vi "Initialize.vi"(8 "error in":errorcluster, 9 "Python Module":path, 10 "Output Folder":path, 11 "G-CLI Runner in":refnum<class "Runner.lvclass">) -> (0 "error out":errorcluster, 3 "G-CLI Runner out":refnum<class "Runner.lvclass">)   [LabVIEW 2026, in "Runner.lvlib" / "Runner.lvclass"]
doc: "Initialize runner."
uses:
  Runner.lvclass
  Runner.lvclass/Runner.ctl
  Interfaces/ILogger/ILogger Messages/Log Msg/Log Msg.lvclass/Log Msg.ctl
  <vilib>/ActorFramework/Message Enqueuer/Message Enqueuer.lvclass/Message Enqueuer.ctl
  <vilib>/ActorFramework/Message Enqueuer/Enqueue.vi
  Interfaces/ILogger/ILogger Messages/Log Msg/Log Msg.lvclass
  <vilib>/ActorFramework/Message Priority Queue/Priority Enqueue.vi
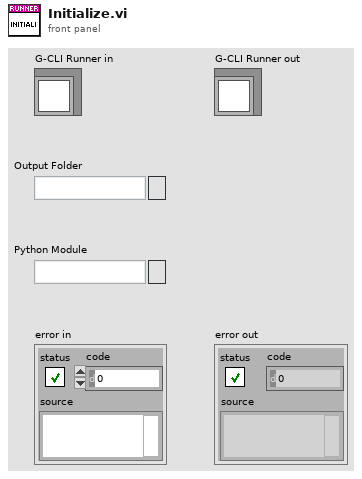
[diagram p1: front panel]
types:
  T1 = typedef "Paths And Strings--cluster.ctl" = cluster{"Project File":path, "Project Folder":path, "Module Name":string}
  T2 = typedef "Log Entry--cluster.ctl" = cluster{"Time":timestamp, "Message":string}
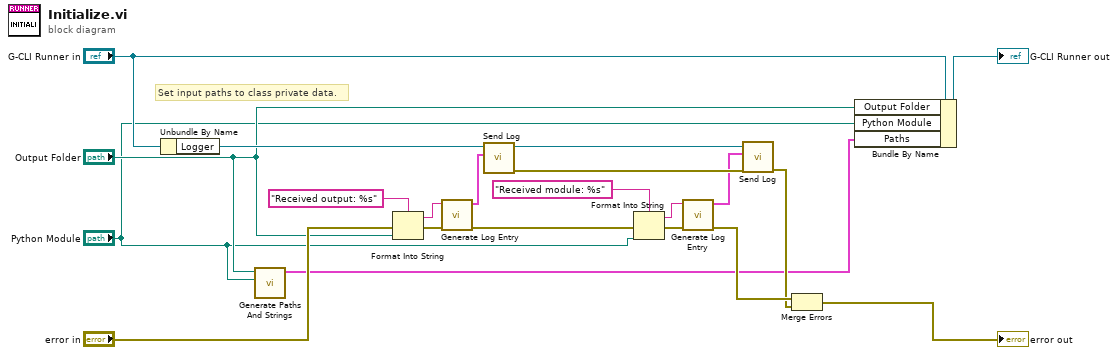
[diagram p0: block diagram]
diagram:
  # "Set input paths to class private data."
  n1 = Unbundle By Name("G-CLI Runner in") -> ("Logger"=w11:refnum<class "Message Enqueuer.lvclass">)
  n2 = call "Generate Paths And Strings.vi"("Python Module"="Python Module", "Output Folder"="Output Folder") -> ("Paths"=w1:T1)  [unwired: 9 in]
  n3 = Format Into String(format string="Received output: %s", error in="error in", "Output Folder") -> (resulting string=w9:string, error out=w16:errorcluster)  [unwired: 1 in]
  n4 = call "Generate Log Entry.vi"("error in"=w16, "Message"=w9) -> ("error out"=w15:errorcluster, "Log Entry"=w8:T2)  [unwired: 8 in]
  n5 = call "Send Log.vi"("Log Entry"=w8, "Message Enqueuer"=w11) -> ("error out"=w20:errorcluster, "Message Enqueuer out"=w5:refnum<class "Message Enqueuer.lvclass">)  [unwired: 8 in]
  n6 = Format Into String(format string="Received module: %s", error in=w15, "Python Module") -> (resulting string=w6:string, error out=w14:errorcluster)  [unwired: 1 in]
  n7 = call "Generate Log Entry.vi"("error in"=w14, "Message"=w6) -> ("error out"=w21:errorcluster, "Log Entry"=w4:T2)  [unwired: 8 in]
  n8 = call "Send Log.vi"("error in (no error)"=w20, "Log Entry"=w4, "Message Enqueuer"=w5) -> ("error out"=w18:errorcluster)  [unwired: 7 in, 1 out]
  n9 = Merge Errors(w21, w18) -> (→"error out":errorcluster)
  n10 = Bundle By Name(cluster="G-CLI Runner in", "Output Folder"="Output Folder", "Python Module"="Python Module", "Paths"=w1) -> (→"G-CLI Runner out":refnum<class "Runner.lvclass">)
